vi "Get Control Terminals.vi"(7 "Indicators?":bool, 8 "error in (no error)":errorcluster, 11 "VI in":refnum<vi>) -> (0 "error out":errorcluster, 2 "Controls":map{string, refnum<vi>}(c390), 3 "VI out":refnum<vi>)   [LabVIEW 2020, in "Mock Class Generator.lvclass"]
uses:
  Mock Class Generator.lvclass
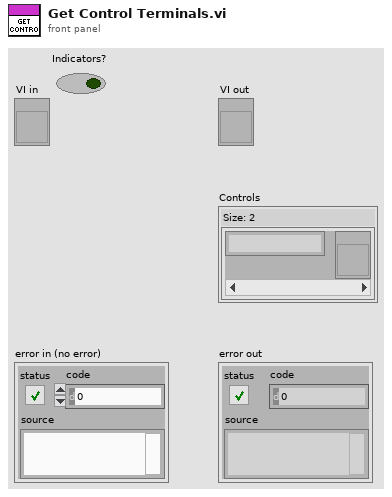
[diagram p1: front panel]
types:
  T1 = enum16{"Invalid Wire Rule", "Required", "Recommended", "Optional", "Dynamic Dispatch"}[]
  T2 = enum16{"Invalid Wire Rule", "Required", "Recommended", "Optional", "Dynamic Dispatch"}
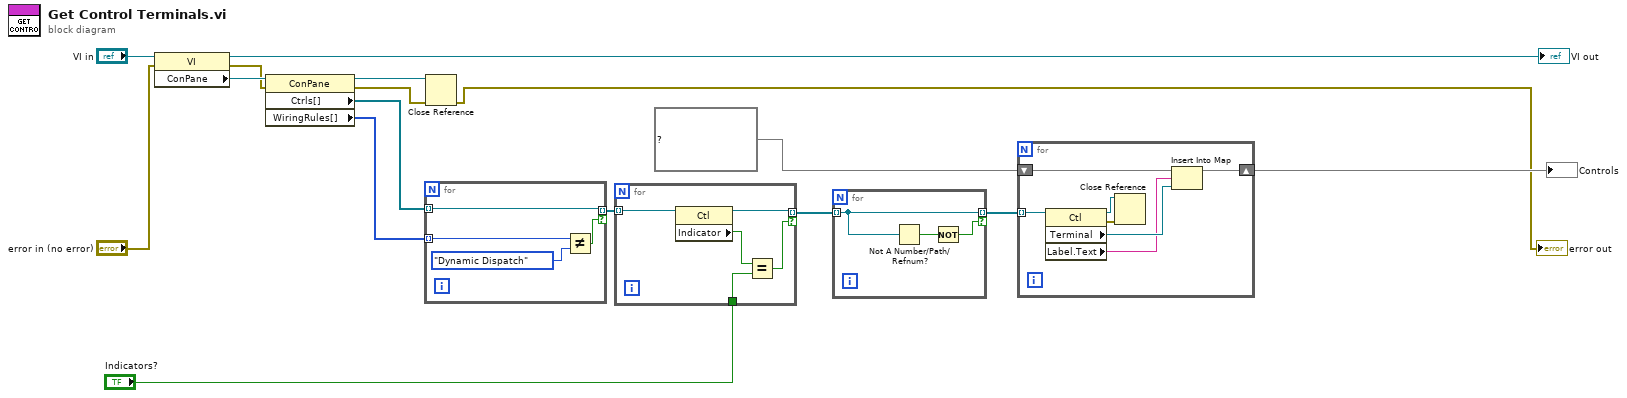
[diagram p0: block diagram]
diagram:
  n1 = property class="VI"(reference="VI in", error in="error in (no error)") -> (reference out=→"VI out":refnum<vi>, error out=w11:errorcluster, "ConPane"=w14:refnum<vi>)
  n2 = property class="ConPane"(reference=w14, error in=w11) -> (reference out=w12:refnum<vi>, error out=w13:errorcluster, "Ctrls[]"=w7:refnum<vi>[], "WiringRules[]"=w6:T1)
  n3 = for {
    tunnel: w7 -> [w18] mode=indexing
    tunnel: w6 -> [w20] mode=indexing
    tunnel: [w18] -> w5 mode=indexing if=w17
    n4 = Not Equal?(x=w20, y=T2."Dynamic Dispatch") -> (x != y?=w17:bool)
  }
  n5 = Close Reference(reference=w12, error in (no error)=w13) -> (error out=→"error out":errorcluster)
  n6 = for {
    tunnel: w5 -> [w25] mode=indexing
    tunnel: [w24] -> w3 mode=indexing if=w21
    tunnel: "Indicators?" -> [w22]
    n7 = property class="Ctl"(reference=w25) -> (reference out=w24:refnum<vi>, "Indicator"=w23:bool)  [unwired: 1 in, 1 out]
    n8 = Equal?(x=w23, y=w22) -> (x = y?=w21:bool)
  }
  n9 = for {
    tunnel: w3 -> [w28] mode=indexing
    tunnel: [w28] -> w2 mode=indexing if=w26
    n10 = Not A Number/Path/Refnum?(number/path/refnum=w28) -> (NaN/Path/Refnum?=w27:bool)
    n11 = Not(x=w27) -> (.not. x?=w26:bool)
  }
  n12 = for {
    shift-right: [w34] -> w8
    shift-left: map{string, refnum<vi>} {} ("map in") -> [w35]
    tunnel: w2 -> [w33] mode=indexing
    n13 = property class="Ctl"(reference=w33) -> (reference out=w30:refnum<vi>, error out=w31:errorcluster, "Terminal"=w32:refnum<vi>, "Label.Text"=w29:string)  [unwired: 1 in]
    n14 = Close Reference(reference=w30, error in (no error)=w31) -> ()  [unwired: 1 out]
    n15 = Insert Into Map(map in=w35, key=w29, value=w32) -> (map out=w34:map{string, refnum<vi>})  [unwired: 2 out]
  }
  "Controls" <- w8
